vi "Create Input Channels.vi"(8 "error in (no error)":errorcluster, 11 "Modbus in":refnum<class "Modbus.lvclass">) -> (0 "error out":errorcluster, 1 "Channels to remove":string[](array[string]), 3 "Modbus out":refnum<class "Modbus.lvclass">)   [LabVIEW 2026, in "Modbus.lvlib" / "Modbus.lvclass"]
uses:
  Modbus.lvclass
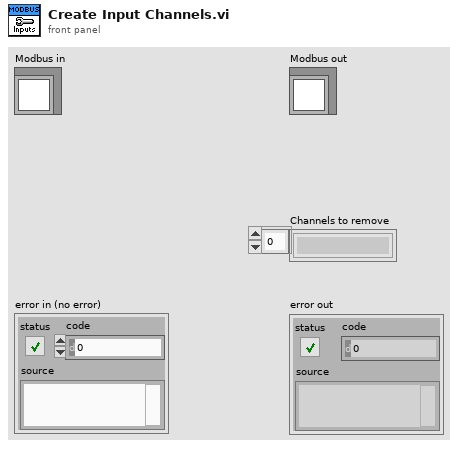
[diagram p1: front panel]
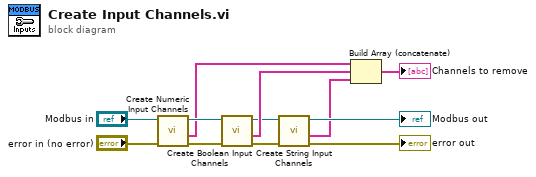
[diagram p0: block diagram]
diagram:
  n1 = call "Create Numeric Input Channels.vi"("error in (no error)"="error in (no error)", "Modbus in"="Modbus in") -> ("error out"=w6:errorcluster, "Channels to remove"=w5:string[], "Modbus out"=w7:refnum<class "Modbus.lvclass">)  [unwired: 7 in]
  n2 = call "Create Boolean Input Channels.vi"("error in (no error)"=w6, "Modbus in"=w7) -> ("error out"=w3:errorcluster, "Channels to remove"=w4:string[], "Modbus out"=w2:refnum<class "Modbus.lvclass">)  [unwired: 7 in]
  n3 = call "Create String Input Channels.vi"("error in (no error)"=w3, "Modbus in"=w2) -> ("error out"=→"error out":errorcluster, "Channels to remove"=w1:string[], "Modbus out"=→"Modbus out":refnum<class "Modbus.lvclass">)  [unwired: 7 in]
  n4 = Build Array (concatenate)(w5, w4, w1) -> (→"Channels to remove":string[])
